vi "mupLib Eval example.vi"() -> ()   [LabVIEW 2015]
uses:
  mupLib/mupLibPath.vi
  mupLib/mupCheckError.vi
  <vilib>/Utility/error.llb/Error Cluster From Error Code.vi
  mupLib/mupLib.lvlib
panel:
  out "x Values":i32[](array[numeric])
  out "error out":errorcluster
  out "Results":dbl[](array[numeric])
  in  "c":dbl=3.0
  in  "Expression":string="a*x^2+b*x+c"
  in  "b":dbl=2.0
  in  "a":dbl=1.0
  # "Constants"
  # "This example demonstrates the basic usage of the mipLib library.\n\n- Enter an expression containing constans \"a\", \"b\", \"c\" and variable \"x\"\n- Enter the values for constants \"a, \"b\" and \"c\".\n- Hit the run button to evaluate the expression for x-values 0 to 9."
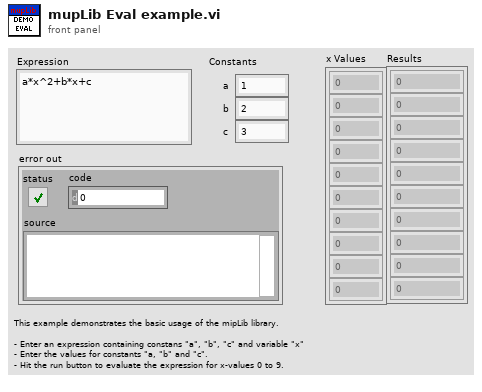
[diagram p1: front panel]
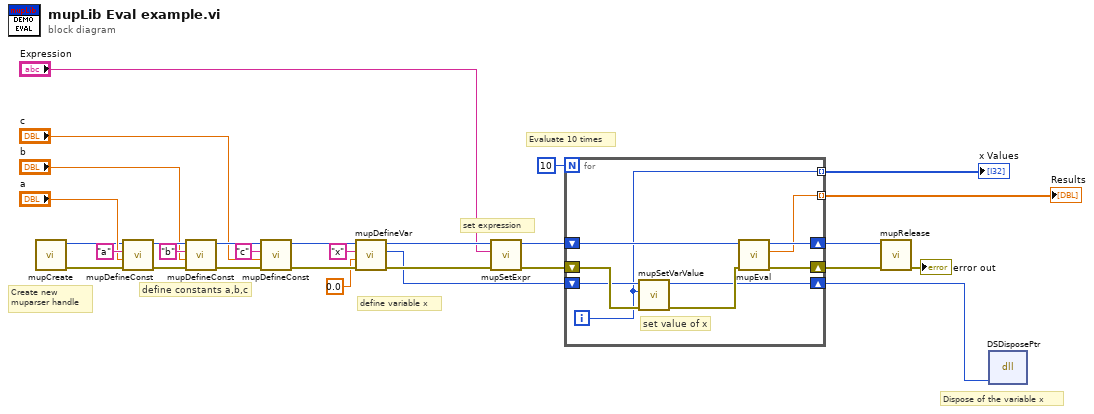
[diagram p0: block diagram]
diagram:
  # "Dispose of the variable x"
  # "Evaluate 10 times"
  # "set expression"
  # "define variable x"
  # "define constants a,b,c"
  # "Create new\nmuparser handle"
  n1 = call "mupCreate.vi"() -> ("error out"=w29:errorcluster, "hParser out"=w3:u64)  [unwired: 10 in]
  n2 = call "mupDefineConst.vi"("error in (no error)"=w29, "Value"="a", "constName"="a", "hParser in"=w3) -> ("error out"=w24:errorcluster, "hParser out"=w25:u64)  [unwired: 6 in]
  n3 = call "mupDefineConst.vi"("error in (no error)"=w24, "Value"="b", "constName"="b", "hParser in"=w25) -> ("error out"=w16:errorcluster, "hParser out"=w17:u64)  [unwired: 6 in]
  n4 = call "mupDefineConst.vi"("error in (no error)"=w16, "Value"="c", "constName"="c", "hParser in"=w17) -> ("error out"=w14:errorcluster, "hParser out"=w13:u64)  [unwired: 6 in]
  n5 = call "mupDefineVar.vi"("error in (no error)"=w14, "initValue"=0.0, "varName"="x", "hParser in"=w13) -> ("error out"=w19:errorcluster, "varAddr"=w9:u64, "hParser out"=w21:u64)  [unwired: 5 in]
  n6 = call "mupSetExpr.vi"("error in (no error)"=w19, "szExpr"="Expression", "muPar in"=w21) -> ("error out"=w11:errorcluster, "muPar out"=w12:u64)  [unwired: 7 in]
  n7 = for {
    N: 10 -> [_]
    shift-right: [w33] -> w6
    shift-left: w12 -> [w36]
    shift-right: [w34] -> w5
    shift-left: w11 -> [w38]
    tunnel: [w32] -> w10 mode=indexing
    shift-right: [w31] -> w8
    shift-left: w9 -> [w37]
    tunnel: [w30] -> w1 mode=indexing
    i -> [w30]
    # "set value of x"
    n8 = call "mupSetVarValue.vi"("error in (no error)"=w38, "varValue"=w30, "varAddr in"=w37) -> ("error out"=w35:errorcluster, "varAddr out"=w31:u64)  [unwired: 7 in]
    n9 = call "mupEval.vi"("error in (no error)"=w35, "hParser in"=w36) -> ("error out"=w34:errorcluster, "result"=w32:dbl, "hParser out"=w33:u64)  [unwired: 7 in]
  }
  "Results" <- w10
  "x Values" <- w1
  n10 = call "mupRelease.vi"("error in (no error)"=w5, "hParser in"=w6) -> ("error out"=→"error out":errorcluster)  [unwired: 9 in]
  n11 = dll-call lib="LabVIEW" fn="DSDisposePtr"("ptr"=w8) -> ()  [unwired: 5 in, 2 out]
